vi "1.fispec_v1_basic.vi"() -> ()   [LabVIEW 2017]
uses:
  <vilib>/Instr/_visa.llb/VISA Configure Serial Port (Instr).vi
panel:
  out "XY Graph":T1(graph)
  out "Waveform Graph":dbl[](graph)
  out "Peak amplitudes":dbl[](array[numeric])
  out "Measured peak wavelengths":dbl[](array[numeric]) format="%.3g"
  in  "Stop":bool
  in  "Integration time (µs)":i32=100000
  in  "FBG channel width (nm)":dbl=2.0 format="%.3g"
  in  "FBG channel wavelength (nm)":dbl[](array[numeric])=[810.0, 812.5, 815.0, 817.5, 820.0, 822.5, 825.0, 827.5, 830.0, 832.5, 835.0, 837.5, 840.0, 842.5, 845.0, 847.5, 850.0, 852.5, 855.0, 857.5, 860.0, 862.5, 865.0, 867.5, 870.0, 872.5, 875.0, 877.5, 880.0, 882.5, 885.0, 887.5] format="%.3g"
  in  "VISA resource name":refnum<visa-resource-name>="COM3" caption="Serial COM port"
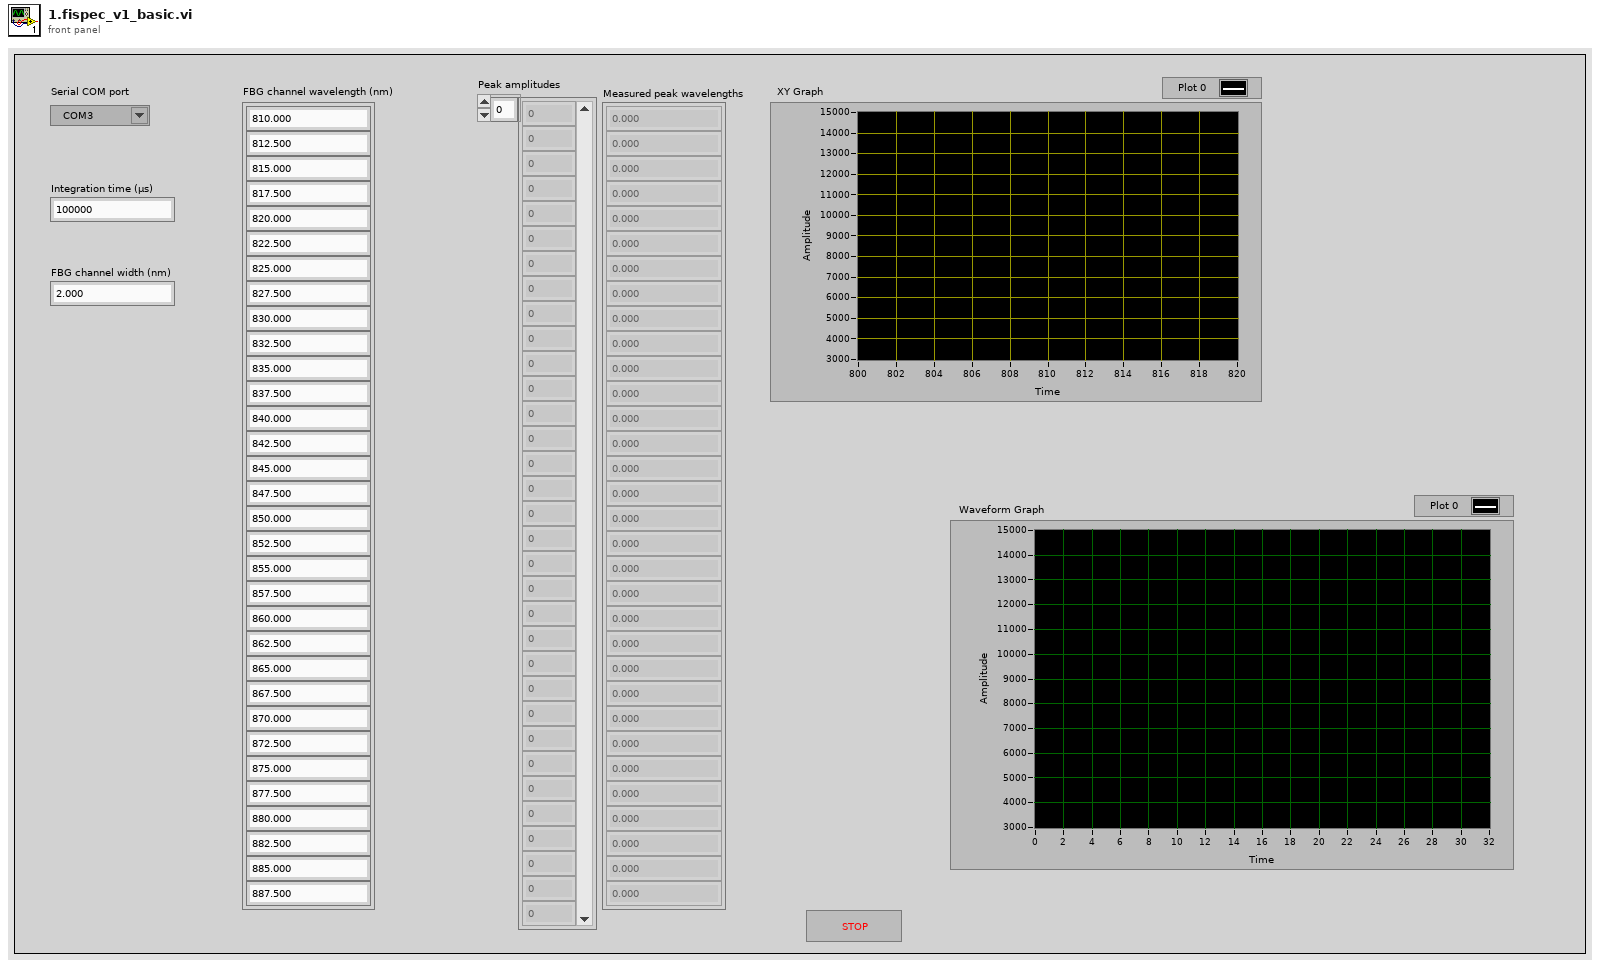
[diagram p1: front panel]
types:
  T1 = cluster{"Peak wavelengths":dbl[], "Peak amplitudes":dbl[]}
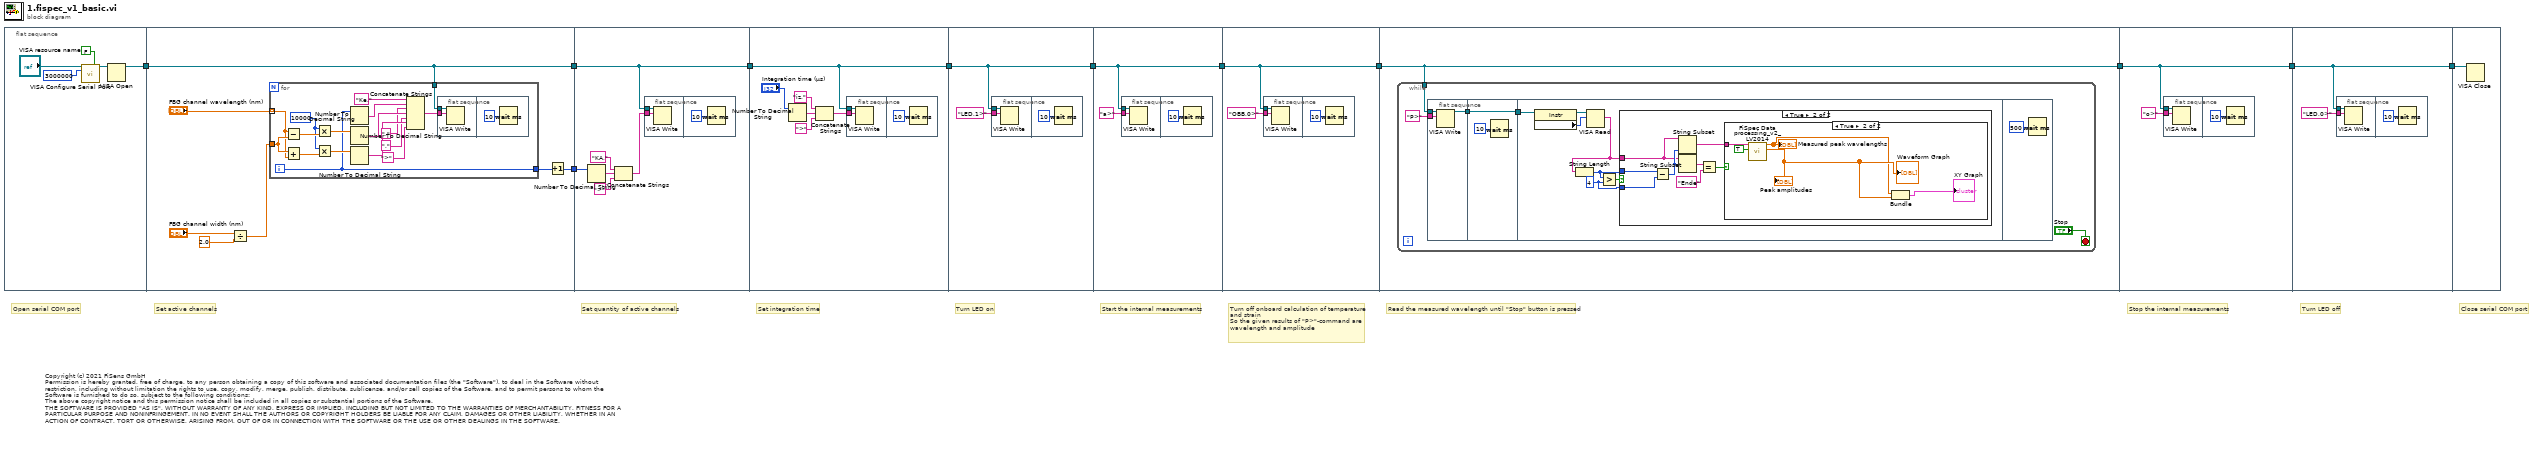
[diagram p0: block diagram]
diagram:
  # "Copyright (c) 2021 FiSens GmbH\nPermission is hereby granted, free of charge, to any person obtaining a copy of this software and associated documentation files (the \"Software\"), to deal in the Software without restriction, including without limitation the rights to use, copy, modify, merge, publish, distribute, sublicense, and/or sell copies of the Software, and to permit persons to whom the Software is furnished to do so, subject to the following conditions:\nThe above copyright notice and this permission notice shall be included in all copies or substantial portions of the Software.\nTHE SOFTWARE IS PROVIDED \"AS IS\", WITHOUT WARRANTY OF ANY KIND, EXPRESS OR IMPLIED, INCLUDING BUT NOT LIMITED TO THE WARRANTIES OF MERCHANTABILITY, FITNESS FOR A PARTICULAR PURPOSE AND NONINFRINGEMENT. IN NO EVENT SHALL THE AUTHORS OR COPYRIGHT HOLDERS BE LIABLE FOR ANY CLAIM, DAMAGES OR OTHER LIABILITY, WHETHER IN AN ACTION OF CONTRACT, TORT OR OTHERWISE, ARISING FROM, OUT OF OR IN CONNECTION WITH THE SOFTWARE OR THE USE OR OTHER DEALINGS IN THE SOFTWARE."
  # "Turn off onboard calculation of temperature and strain\nSo the given results of \"P>\"-command are wavelength and amplitude"
  # "Close serial COM port"
  # "Turn LED off"
  # "Stop the internal measurements"
  # "Read the measured wavelength until \"Stop\" button is pressed"
  # "Start the internal measurements"
  # "Turn LED on"
  # "Set integration time"
  # "Open serial COM port"
  # "Set quantity of active channels"
  # "Set active channels"
  n1 = flat-sequence {
    tunnel: [w13] -> w9
    tunnel: [w19] -> w11
    tunnel: [w17] -> w10
    tunnel: w9 -> [w19]
    tunnel: w11 -> [w49]
    tunnel: w10 -> [w45]
    tunnel: [w49] -> w8
    tunnel: w8 -> [w53]
    tunnel: [w53] -> w7
    tunnel: w7 -> [w63]
    tunnel: [w63] -> w6
    tunnel: w6 -> [w67]
    tunnel: [w67] -> w2
    tunnel: w2 -> [w72]
    tunnel: [w72] -> w1
    tunnel: w1 -> [w77]
    tunnel: [w77] -> w5
    tunnel: w5 -> [w109]
    tunnel: [w109] -> w4
    tunnel: w4 -> [w114]
    tunnel: [w114] -> w3
    tunnel: w3 -> [w119]
    frame #0 {
      n2 = call-poly "VISA Configure Serial Port"("VISA resource name"="VISA resource name", "Enable Termination\nChar (T)"=FALSE ("Enable Termination\nChar (T)"), "baud rate (9600)"=u32 3000000) -> ("VISA resource name out"=w16:refnum<visa-resource-name>)  [unwired: 11 in, 1 out]
      n3 = VISA Open(VISA resource name=w16) -> (VISA resource name=w13:refnum<visa-resource-name>)  [unwired: 4 in, 1 out]
    }
    frame #1 {
      n4 = Divide(x="FBG channel width (nm)", y=2.0) -> (x/y=w20:dbl)
      n5 = for {
        tunnel: "FBG channel wavelength (nm)" -> [w38] mode=indexing
        tunnel: w19 -> [w40]
        tunnel: w20 -> [w39]
        tunnel: [w24] -> w18
        i -> [w24]
        w35 = 10000
        n6 = Subtract(x=w38, y=w39) -> (x-y=w37:dbl)
        n7 = Add(x=w39, y=w38) -> (x+y=w36:dbl)
        n8 = Multiply(x=w35, y=w37) -> (x*y=w33:dbl)
        n9 = Multiply(x=w35, y=w36) -> (x*y=w34:dbl)
        n10 = Number To Decimal String(number=w24) -> (decimal integer string=w31:string)  [unwired: 1 in]
        n11 = Number To Decimal String(number=w33) -> (decimal integer string=w30:string)  [unwired: 1 in]
        n12 = Number To Decimal String(number=w34) -> (decimal integer string=w29:string)  [unwired: 1 in]
        n13 = Concatenate Strings("Ke," ("String"), w31, "," ("String"), w30, "," ("String"), w29, ">" ("String")) -> (w25:string)
        n14 = flat-sequence {
          tunnel: w40 -> [w42]
          tunnel: w25 -> [w41]
          frame #0 {
            n15 = VISA Write(VISA resource name=w42, write buffer=w41) -> ()  [unwired: 1 in, 3 out]
          }
          frame #1 {
            n16 = Wait (ms)(milliseconds to wait=u32 10 ("Zu wartende ms")) -> ()  [unwired: 1 out]
          }
        }
      }
      n17 = Increment(x=w18) -> (x+1=w17:i32)
    }
    frame #2 {
      n18 = Number To Decimal String(number=w45) -> (decimal integer string=w46:string)  [unwired: 1 in]
      n19 = Concatenate Strings("KA," ("String"), w46, ">" ("String")) -> (w44:string)
      n20 = flat-sequence {
        tunnel: w49 -> [w51]
        tunnel: w44 -> [w50]
        frame #0 {
          n21 = VISA Write(VISA resource name=w51, write buffer=w50) -> ()  [unwired: 1 in, 3 out]
        }
        frame #1 {
          n22 = Wait (ms)(milliseconds to wait=u32 10 ("Zu wartende ms")) -> ()  [unwired: 1 out]
        }
      }
    }
    frame #3 {
      n23 = Number To Decimal String(number="Integration time (µs)") -> (decimal integer string=w58:string)  [unwired: 1 in]
      n24 = Concatenate Strings("iz," ("String"), w58, ">" ("String")) -> (w55:string)
      n25 = flat-sequence {
        tunnel: w53 -> [w60]
        tunnel: w55 -> [w59]
        frame #0 {
          n26 = VISA Write(VISA resource name=w60, write buffer=w59) -> ()  [unwired: 1 in, 3 out]
        }
        frame #1 {
          n27 = Wait (ms)(milliseconds to wait=u32 10 ("Zu wartende ms")) -> ()  [unwired: 1 out]
        }
      }
    }
    frame #4 {
      n28 = flat-sequence {
        tunnel: w63 -> [w65]
        tunnel: "LED,1>" ("String") -> [w64]
        frame #0 {
          n29 = VISA Write(VISA resource name=w65, write buffer=w64) -> ()  [unwired: 1 in, 3 out]
        }
        frame #1 {
          n30 = Wait (ms)(milliseconds to wait=u32 10 ("Zu wartende ms")) -> ()  [unwired: 1 out]
        }
      }
    }
    frame #5 {
      n31 = flat-sequence {
        tunnel: w67 -> [w70]
        tunnel: "a>" ("String") -> [w69]
        frame #0 {
          n32 = VISA Write(VISA resource name=w70, write buffer=w69) -> ()  [unwired: 1 in, 3 out]
        }
        frame #1 {
          n33 = Wait (ms)(milliseconds to wait=u32 10 ("Zu wartende ms")) -> ()  [unwired: 1 out]
        }
      }
    }
    frame #6 {
      n34 = flat-sequence {
        tunnel: w72 -> [w75]
        tunnel: "OBB,0>" ("String") -> [w74]
        frame #0 {
          n35 = VISA Write(VISA resource name=w75, write buffer=w74) -> ()  [unwired: 1 in, 3 out]
        }
        frame #1 {
          n36 = Wait (ms)(milliseconds to wait=u32 10 ("Zu wartende ms")) -> ()  [unwired: 1 out]
        }
      }
    }
    frame #7 {
      n37 = while {
        tunnel: w77 -> [w81]
        stop <- "Stop" stop-if-true
        n38 = flat-sequence {
          tunnel: w81 -> [w85]
          tunnel: "P>" ("String") -> [w84]
          tunnel: [w83] -> w78
          tunnel: [w86] -> w79
          tunnel: w78 -> [w86]
          tunnel: w79 -> [w94]
          frame #0 {
            n39 = VISA Write(VISA resource name=w85, write buffer=w84) -> (VISA resource name out=w83:refnum<visa-resource-name>)  [unwired: 1 in, 2 out]
          }
          frame #1 {
            n40 = Wait (ms)(milliseconds to wait=u32 10 ("Zu wartende ms")) -> ()  [unwired: 1 out]
          }
          frame #2 {
            w89 = 4 ("y")
            n41 = property class="Instr"(reference=w94) -> (reference out=w93:refnum<visa-resource-name>, "Serial Settings:Number of Bytes at Serial Port"=w92:u32)  [unwired: 1 in, 1 out]
            n42 = VISA Read(VISA resource name=w93, byte count=w92) -> (read buffer=w88:string)  [unwired: 1 in, 3 out]
            n43 = String Length(string=w88) -> (length=w90:i32)
            n44 = Greater?(x=w90, y=w89) -> (0:w91:bool)
            n45 = case shown="True" w91 {
              tunnel: w88 -> [_ w99]
              tunnel: w90 -> [_ w97]
              tunnel: w89 -> [_ w96]
              frame False {
              }
              frame True {
                n46 = Subtract(x=w97, y=w96) -> (x-y=w100:i32)
                n47 = String Subset(string=w99, length (rest)=w100) -> (substring=w98:string)  [unwired: 1 in]
                n48 = String Subset(string=w99, offset (0)=w100) -> (substring=w102:string)  [unwired: 1 in]
                n49 = Equal?(x=w102, y="Ende") -> (x = y?=w95:bool)
                n50 = case shown="True" w95 {
                  tunnel: w98 -> [_ w107]
                  frame False {
                  }
                  frame True {
                    n51 = call "FiSpec Data processing_v2_LV2014.vi"("Onboard peak detection"=TRUE, "Data string (without \"Ende\")"=w107) -> ("Peak amplitudes"=w105:dbl[], "Peak wavelengths"=w104:dbl[])  [unwired: 4 in, 4 out]
                    "Measured peak wavelengths" <- w104
                    "Peak amplitudes" <- w105
                    "Waveform Graph" <- w105
                    n52 = Bundle("Peak wavelengths"=w104, "Peak amplitudes"=w105) -> (→"XY Graph":T1)  [unwired: 1 in]
                  }
                }
              }
            }
          }
          frame #3 {
            n53 = Wait (ms)(milliseconds to wait=u32 500 ("Zu wartende ms")) -> ()  [unwired: 1 out]
          }
        }
      }
    }
    frame #8 {
      n54 = flat-sequence {
        tunnel: w109 -> [w112]
        tunnel: "o>" ("String") -> [w111]
        frame #0 {
          n55 = VISA Write(VISA resource name=w112, write buffer=w111) -> ()  [unwired: 1 in, 3 out]
        }
        frame #1 {
          n56 = Wait (ms)(milliseconds to wait=u32 10 ("Zu wartende ms")) -> ()  [unwired: 1 out]
        }
      }
    }
    frame #9 {
      n57 = flat-sequence {
        tunnel: w114 -> [w117]
        tunnel: "LED,0>" ("String") -> [w116]
        frame #0 {
          n58 = VISA Write(VISA resource name=w117, write buffer=w116) -> ()  [unwired: 1 in, 3 out]
        }
        frame #1 {
          n59 = Wait (ms)(milliseconds to wait=u32 10 ("Zu wartende ms")) -> ()  [unwired: 1 out]
        }
      }
    }
    frame #10 {
      n60 = VISA Close(VISA resource name=w119) -> ()  [unwired: 1 in, 1 out]
    }
  }
